vi "SetWindowRgn Wrapper Template.vi"(0 "hWnd":u64, 5 "hRgn":u64, 7 "bRedraw":i32=1, 11 "error in":errorcluster) -> (4 "return value":i32, 15 "error out":errorcluster)   [LabVIEW 2020]
doc: "Sets the window region of hWnd - the part of the window the system draws on screen - through user32.dll SetWindowRgn (stdcall, called in any thread). An empty region (gdi32 CreateRectRgn.vi 0, 0, 0, 0) makes the window invisible on screen, also while its owner animates its opacity; it stays open, functional and capturable with PrintWindow (measured on a LabVIEW menu). hRgn 0 removes the region. After a successful call the system owns hRgn; do not delete it. return value is non-zero on success. When error in carries an error the DLL is not called. Generated by tools\\Build Win32 Wrappers.vi - do not edit by hand, rebuild it."
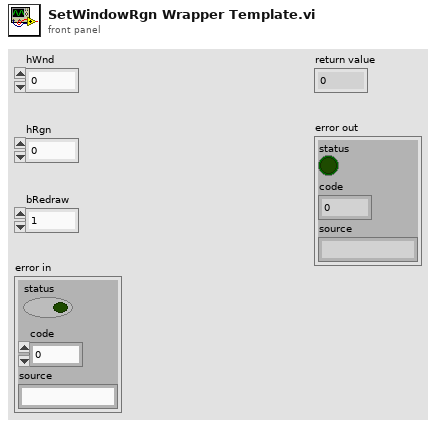
[diagram p1: front panel]
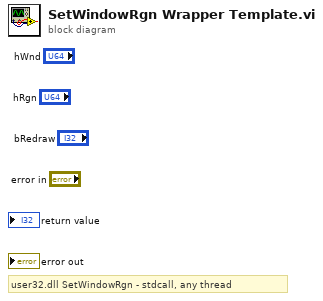
[diagram p0: block diagram]
diagram:
  # "user32.dll SetWindowRgn - stdcall, any thread"
